vi "外观.vi"(0 "Data In":T6 caption="数据输入", 2 "Display State In":T3 caption="显示状态输入", 3 "Container State":T5 caption="容器状态") -> (6 "Data Out":T6 caption="数据输出", 7 "Display State Out":T3 caption="显示状态输出", 8 "Action":T2 caption="动作")   [LabVIEW 2025, in "XButton.lvlib" / "button3.xctl"]
uses:
  button3.xctl
  <vilib>/_xctls/Container State.ctl
  helper loop Events.ctl
  move event.ctl
  <vilib>/_xctls/Action.ctl
  button.ctl
  <vilib>/_xctls/XControlSupport.lvlib
panel:
  in  "确定按钮":T1
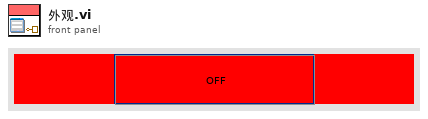
[diagram p1: front panel]
types:
  T1 = typedef "XButton.lvlib/button3.xctl/button.ctl" = bool
  T2 = typedef "XControlSupport.lvlib/Action.ctl" = cluster{"Data Changed?":bool, "State Changed?":bool, "Action Name":string}
  T3 = typedef "XButton.lvlib/button3.xctl/状态.ctl" = cluster{"Numeric":dbl, "调用方窗格颜色":u32, "按钮颜色":u32, "helper loop data":T4, "布尔文本":string, "字体颜色":u32, "字号":u32, "动效风格":enum16{"风格一", "风格二", "风格三", "风格四"}, "已隐藏不需要遮罩层":bool, "已初始化遮罩层位置":bool}
  T4 = typedef "XButton.lvlib/button3.xctl/helper loop Events.ctl" = cluster{"停止用户事件":refnum<user-event>, "修饰1move用户事件输出":refnum<user-event>, "修饰2move用户事件输出":refnum<user-event>}
  T5 = typedef "XControlSupport.lvlib/Container State.ctl" = cluster{"Indicator?":bool, "Run Mode?":bool, " Refnum":refnum<vi>}
  T6 = typedef "XButton.lvlib/button3.xctl/数据.ctl" = bool
  T7 = typedef "XButton.lvlib/button3.xctl/move event.ctl" = cluster{"Decor引用句柄":refnum<vi>, "b":dbl, "c":dbl, "动效风格":enum16{"风格一", "风格二", "风格三", "风格四"}, "方向(T:离开/F:进入)":bool}
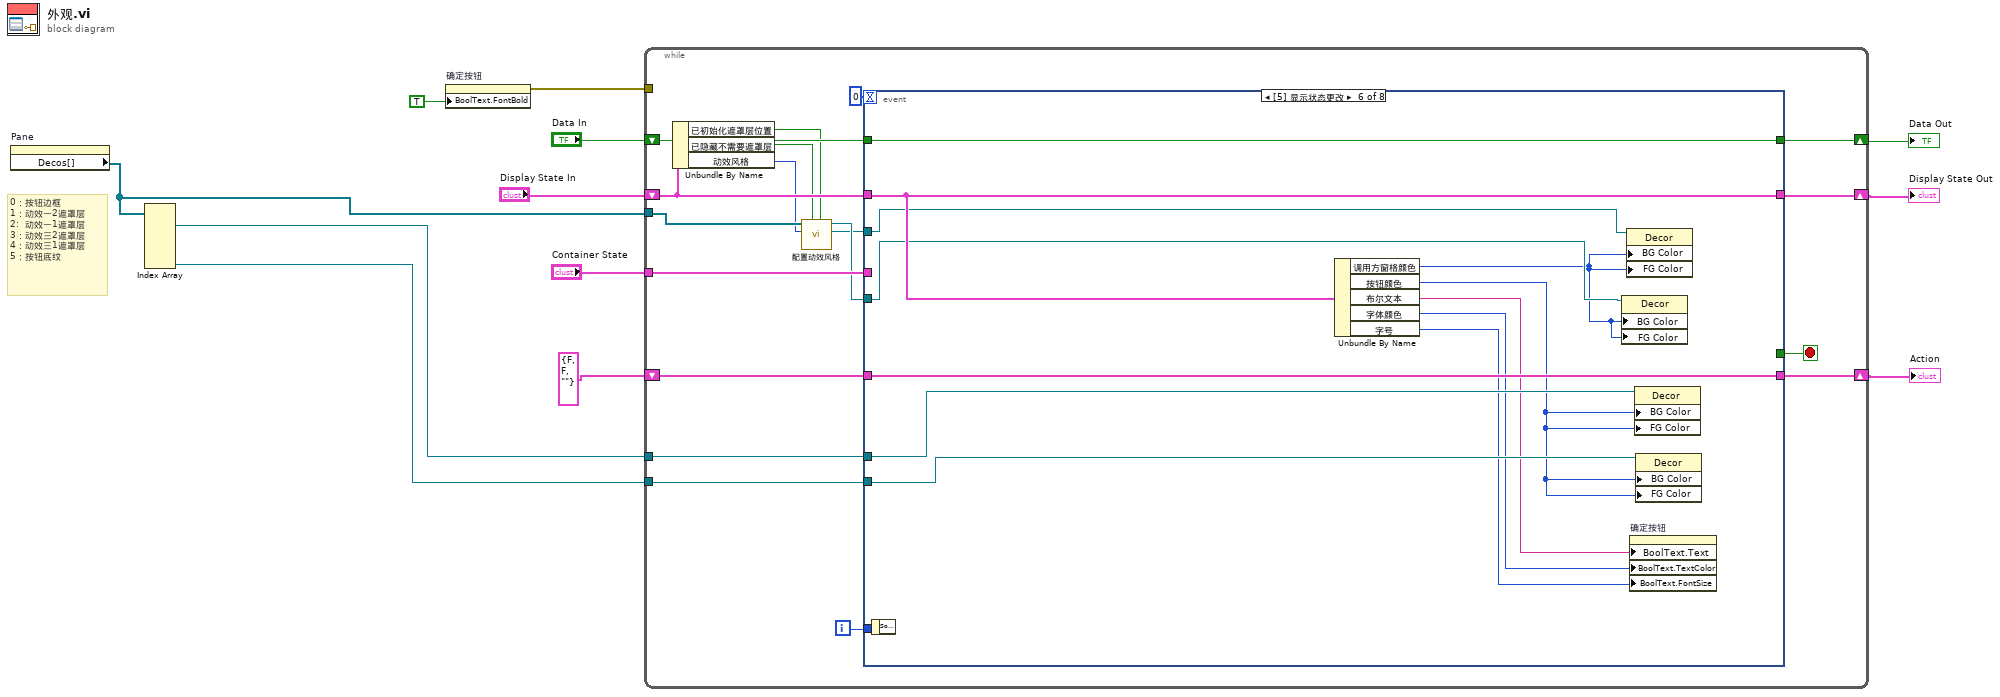
[diagram p0: block diagram]
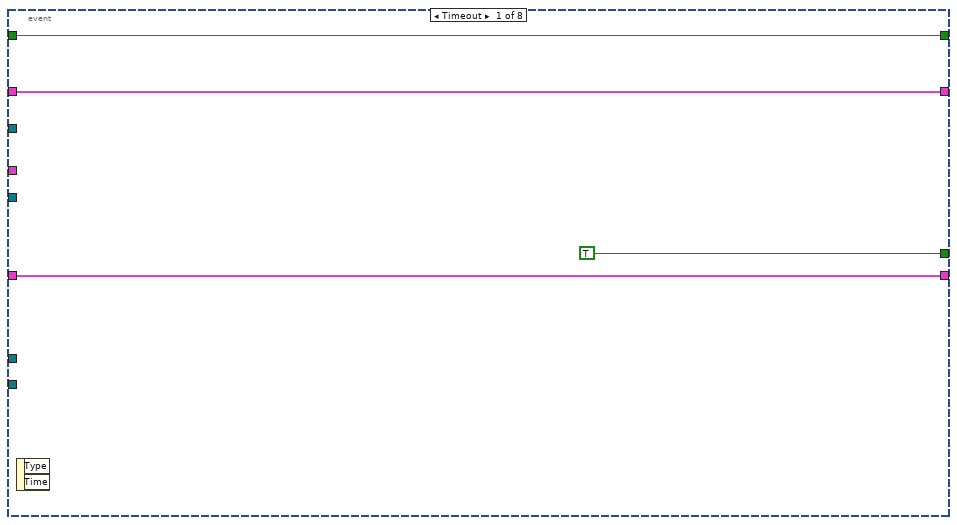
[diagram p2: hidden frame]
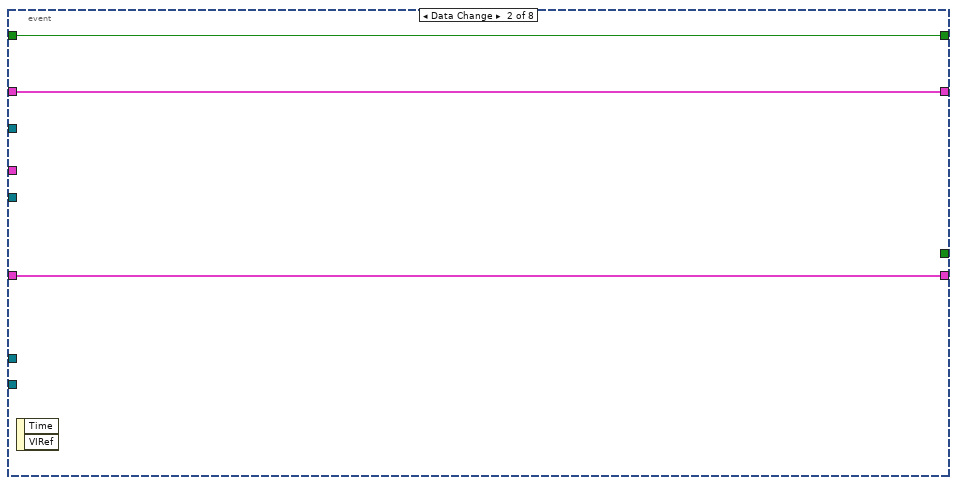
[diagram p3: hidden frame]
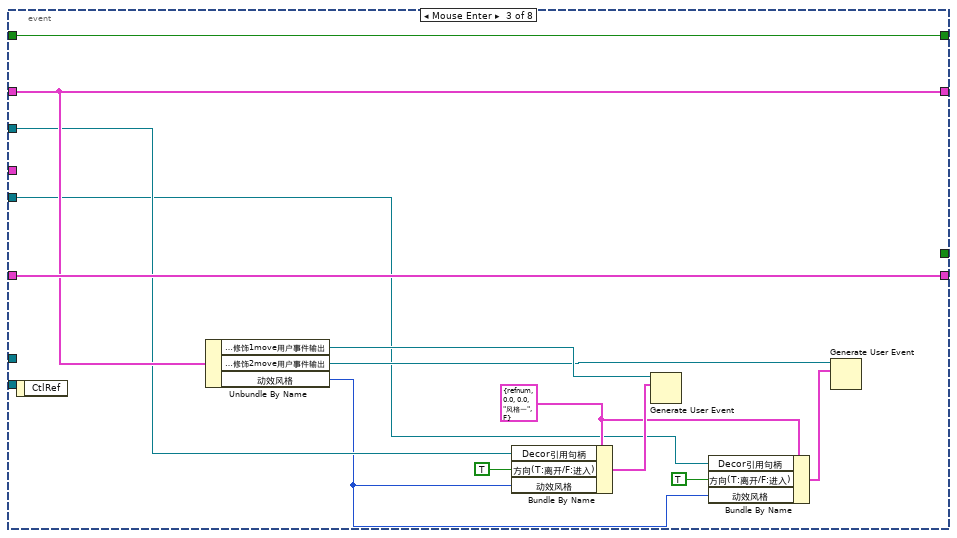
[diagram p4: hidden frame]
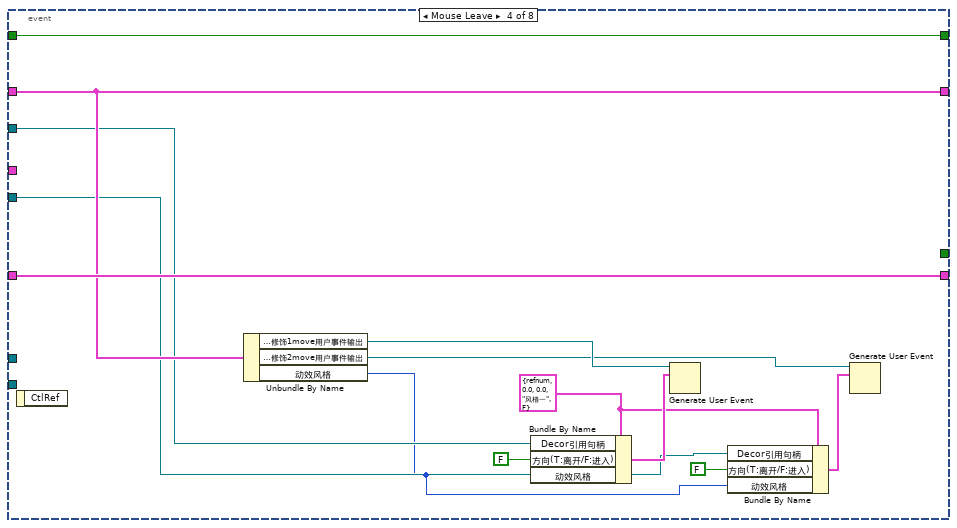
[diagram p5: hidden frame]
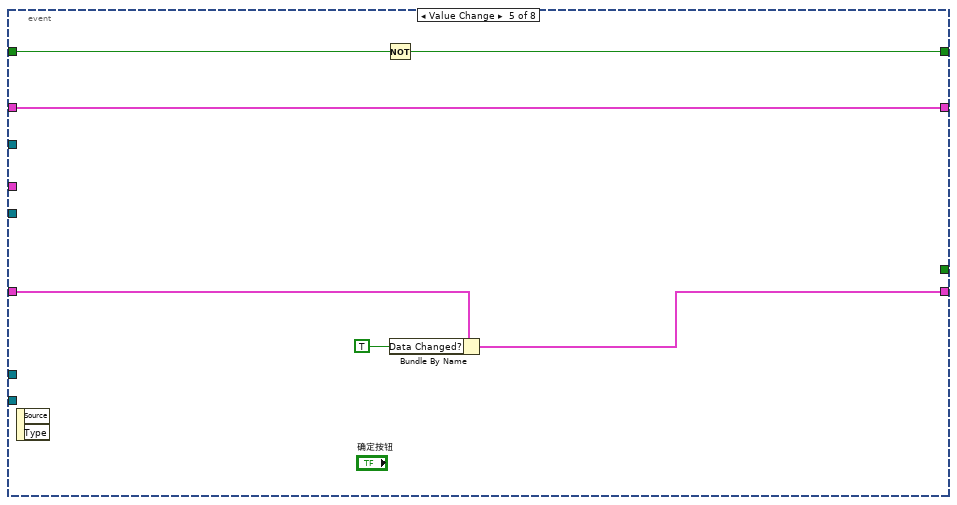
[diagram p6: hidden frame]
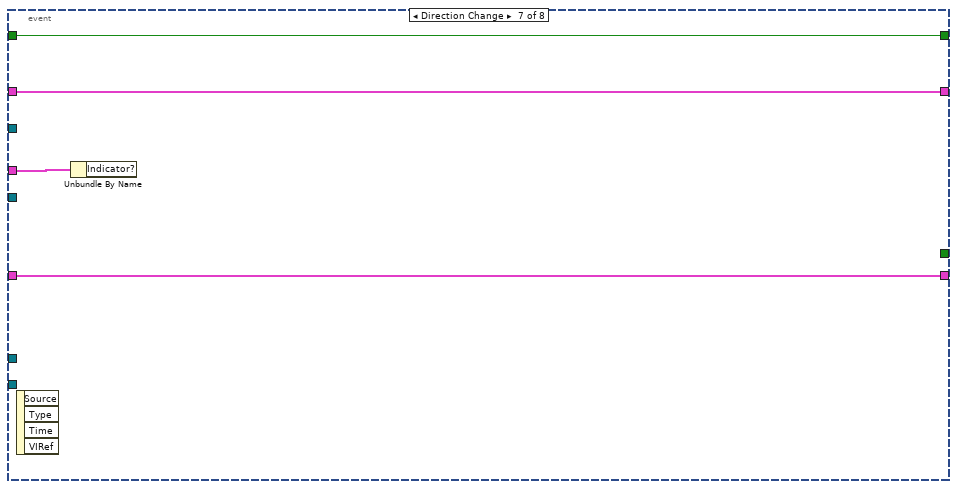
[diagram p7: hidden frame]
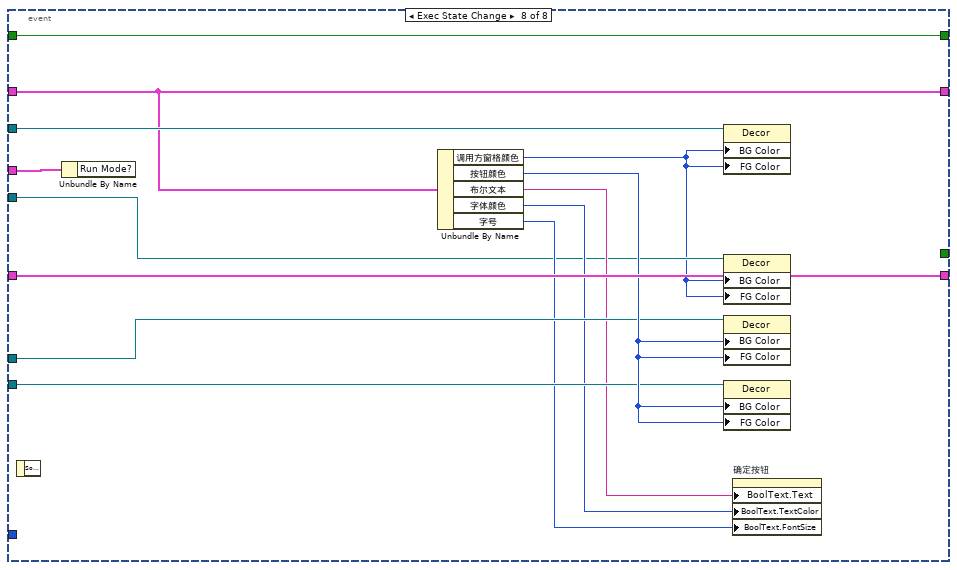
[diagram p8: hidden frame]
diagram:
  # "0：按钮边框\n1：动效一2遮罩层\n2:  动效一1遮罩层\n3：动效三2遮罩层\n4：动效三1遮罩层\n5：按钮底纹"
  n1 = property on="Pane" class="Pane"() -> ("Decos[]"=w2:refnum<vi>[])  [unwired: 2 in, 2 out]
  n2 = Index Array(array=w2) -> (element #1=w4:refnum<vi>, element #6=w5:refnum<vi>)  [unwired: 6 in, 4 out]
  n3 = property on="确定按钮" class="Bool"("BoolText.FontBold"=TRUE ("布尔文本.字体:粗体")) -> (error out=w7:errorcluster)  [unwired: 2 in, 1 out]
  n4 = while {
    shift-right: [w13] -> w3
    shift-left: "Display State In" -> [w19]
    tunnel: "Container State" -> [w28]
    shift-right: [w26] -> w12
    shift-left: "Data In" -> [w27]
    shift-right: [w24] -> w9
    shift-left: T2 {"Data Changed?"=FALSE, "State Changed?"=FALSE, "Action Name"=""} ("Action") -> [w25]
    tunnel: w4 -> [w22]
    tunnel: w5 -> [w21]
    tunnel: w7 -> [_]
    tunnel: w2 -> [w20]
    i -> [w23]
    stop <- w30 stop-if-true
    n5 = Unbundle By Name(w19) -> ("已初始化遮罩层位置"=w14:bool, "已隐藏不需要遮罩层"=w15:bool, "动效风格"=w18:enum16{"风格一", "风格二", "风格三", "风格四"})
    n6 = call "配置动效风格.vi"("已初始化"=w14, "已隐藏不需要的遮罩层"=w15, "动效风格"=w18, "遮罩层引用"=w20) -> ("动效2引用"=w16:refnum<vi>, "动效1引用"=w17:refnum<vi>)  [unwired: 5 in, 1 out]
    n7 = event "事件结构" shown="[5] 显示状态更改" {
      selector: _ -> [_ _ _ _ _ _ _ _]
      dyn-events: _ -> [_ _ _ _ _ _ _ _]
      timeout: 0 -> [_ _ _ _ _ _ _ _]
      tunnel: w19 -> [w33 w35 w43 w57 w69 w79 w84 w87]
      tunnel: [w33 w35 w43 w57 w69 w79 w84 w87] -> w13
      tunnel: [TRUE _ _ _ _ _ _ _] -> w30
      tunnel: w28 -> [_ _ _ _ _ _ w85 w98]
      tunnel: w27 -> [w32 w36 w50 w63 w68 w81 w83 w97]
      tunnel: [w32 w36 w50 w63 w67 w81 w83 w97] -> w26
      tunnel: [w34 w37 w49 w62 w65 w80 w82 w96] -> w24
      tunnel: w25 -> [w34 w37 w49 w62 w66 w80 w82 w96]
      tunnel: w16 -> [_ _ w42 w55 _ w72 _ w89]
      tunnel: w17 -> [_ _ w41 w54 _ w71 _ w88]
      tunnel: w23 -> [_ _ _ _ _ _ _ _]
      tunnel: w22 -> [_ _ _ _ _ w78 _ w94]
      tunnel: w21 -> [_ _ _ _ _ w77 _ w93]
      event Timeout {
        n8 = event-data() -> ()  [unwired: 1 in, 2 out]
      }
      event Data Change {
        n9 = event-data() -> ()  [unwired: 1 in, 2 out]
      }
      event Mouse Enter {
        w46 = T7 {"Decor引用句柄"=refnum, "b"=0.0, "c"=0.0, "动效风格"=enum."风格一", "方向(T:离开/F:进入)"=FALSE} ("事件数据")
        n10 = event-data() -> ()  [unwired: 1 in, 1 out]
        n11 = Unbundle By Name(w43) -> ("helper loop data.修饰1move用户事件输出"=w48:refnum<user-event>, "helper loop data.修饰2move用户事件输出"=w44:refnum<user-event>, "动效风格"=w40:enum16{"风格一", "风格二", "风格三", "风格四"})
        n12 = Bundle By Name(cluster=w46, "Decor引用句柄"=w42, "方向(T:离开/F:进入)"=TRUE, "动效风格"=w40) -> (w47:T7)
        n13 = Generate User Event(user event=w48, event data cluster=w47) -> ()  [unwired: 2 in, 2 out]
        n14 = Bundle By Name(cluster=w46, "Decor引用句柄"=w41, "方向(T:离开/F:进入)"=TRUE, "动效风格"=w40) -> (w45:T7)
        n15 = Generate User Event(user event=w44, event data cluster=w45) -> ()  [unwired: 2 in, 2 out]
      }
      event Mouse Leave {
        w59 = T7 {"Decor引用句柄"=refnum, "b"=0.0, "c"=0.0, "动效风格"=enum."风格一", "方向(T:离开/F:进入)"=FALSE} ("事件数据")
        n16 = event-data() -> ()  [unwired: 1 in, 1 out]
        n17 = Unbundle By Name(w57) -> ("helper loop data.修饰1move用户事件输出"=w61:refnum<user-event>, "helper loop data.修饰2move用户事件输出"=w56:refnum<user-event>, "动效风格"=w53:enum16{"风格一", "风格二", "风格三", "风格四"})
        n18 = Bundle By Name(cluster=w59, "Decor引用句柄"=w55, "方向(T:离开/F:进入)"=FALSE, "动效风格"=w53) -> (w60:T7)
        n19 = Generate User Event(user event=w61, event data cluster=w60) -> ()  [unwired: 2 in, 2 out]
        n20 = Bundle By Name(cluster=w59, "Decor引用句柄"=w54, "方向(T:离开/F:进入)"=FALSE, "动效风格"=w53) -> (w58:T7)
        n21 = Generate User Event(user event=w56, event data cluster=w58) -> ()  [unwired: 2 in, 2 out]
      }
      event Value Change {
        n22 = event-data() -> ()  [unwired: 1 in, 2 out]
        n23 = Not(x=w68) -> (.not. x?=w67:T6)
        n24 = Bundle By Name(cluster=w66, "Data Changed?"=TRUE) -> (w65:T2)
      }
      event Display State Change {
        n25 = event-data() -> ()  [unwired: 1 in, 1 out]
        n26 = Unbundle By Name(w79) -> ("调用方窗格颜色"=w70:u32, "按钮颜色"=w76:u32, "布尔文本"=w75:string, "字体颜色"=w74:u32, "字号"=w73:u32)
        n27 = property class="Decor"(reference=w71, "BG Color"=w70, "FG Color"=w70) -> ()  [unwired: 1 in, 2 out]
        n28 = property class="Decor"(reference=w72, "BG Color"=w70, "FG Color"=w70) -> ()  [unwired: 1 in, 2 out]
        n29 = property on="确定按钮" class="Bool"("BoolText.Text"=w75, "BoolText.TextColor"=w74, "BoolText.FontSize"=w73) -> ()  [unwired: 2 in, 2 out]
        n30 = property class="Decor"(reference=w78, "BG Color"=w76, "FG Color"=w76) -> ()  [unwired: 1 in, 2 out]
        n31 = property class="Decor"(reference=w77, "BG Color"=w76, "FG Color"=w76) -> ()  [unwired: 1 in, 2 out]
      }
      event Direction Change {
        n32 = event-data() -> ()  [unwired: 1 in, 4 out]
        n33 = Unbundle By Name(w85) -> ()  [unwired: 1 out]
      }
      event Exec State Change {
        n34 = event-data() -> ()  [unwired: 1 in, 1 out]
        n35 = Unbundle By Name(w98) -> ()  [unwired: 1 out]
        n36 = Unbundle By Name(w87) -> ("调用方窗格颜色"=w86:u32, "按钮颜色"=w95:u32, "布尔文本"=w92:string, "字体颜色"=w91:u32, "字号"=w90:u32)
        n37 = property class="Decor"(reference=w89, "BG Color"=w86, "FG Color"=w86) -> ()  [unwired: 1 in, 2 out]
        n38 = property class="Decor"(reference=w88, "BG Color"=w86, "FG Color"=w86) -> ()  [unwired: 1 in, 2 out]
        n39 = property class="Decor"(reference=w94, "BG Color"=w95, "FG Color"=w95) -> ()  [unwired: 1 in, 2 out]
        n40 = property class="Decor"(reference=w93, "BG Color"=w95, "FG Color"=w95) -> ()  [unwired: 1 in, 2 out]
        n41 = property on="确定按钮" class="Bool"("BoolText.Text"=w92, "BoolText.TextColor"=w91, "BoolText.FontSize"=w90) -> ()  [unwired: 2 in, 2 out]
      }
    }
  }
  "Display State Out" <- w3
  "Data Out" <- w12
  "Action" <- w9
